vi "Get Dependencies.vi"(8 "error in":errorcluster, 9 "Entire Hierarchy":bool, 10 "File Path":path, 11 "LV File Creator in":refnum<class "LV File Creator.lvclass">) -> (0 "error out":errorcluster, 2 "Dependencies":path[](array[path]), 3 "LV File Creator out":refnum<class "LV File Creator.lvclass">)   [LabVIEW 2026, in "LV File Creator.lvclass"]
doc: "This VI determines dependencies of a LabVIEW file."
uses:
  LV File Creator.lvclass
  LV File Creator.lvclass/LV File Creator.ctl
  Interfaces/ILogger/ILogger Messages/Log Msg/Log Msg.lvclass
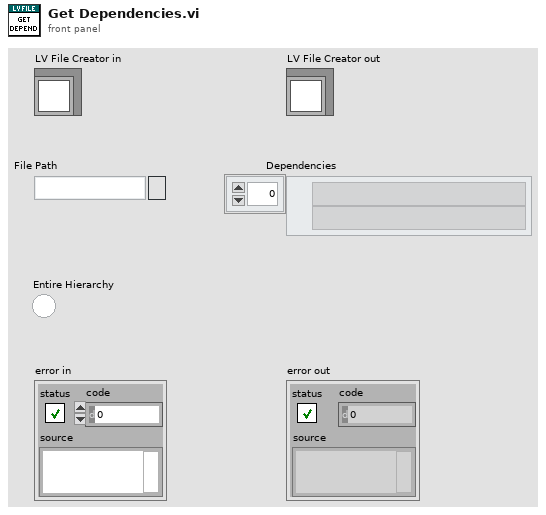
[diagram p1: front panel]
types:
  T1 = enum8{"Only include commented out diagrams if diagram already loaded", "Never include commented out diagrams", "Always include commented out diagrams"}
  T2 = typedef "Log Entry--cluster.ctl" = cluster{"Time":timestamp, "Message":string}
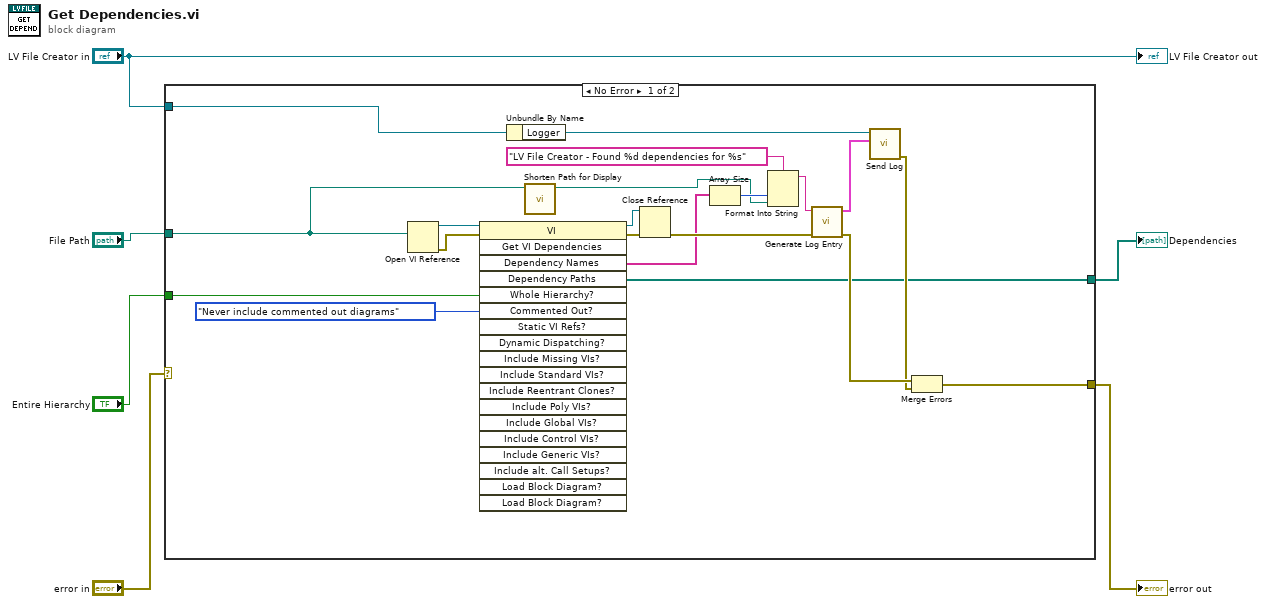
[diagram p0: block diagram]
diagram:
  n1 = case shown="No Error" "error in" {
    selector: "error in" -> [_ w27]
    tunnel: "LV File Creator in" -> [w20 _]
    tunnel: "File Path" -> [w14 _]
    tunnel: [w22 w27] -> w5
    tunnel: [w9 _] -> w2
    tunnel: "Entire Hierarchy" -> [w7 _]
    frame No Error {
      n2 = Open VI Reference(vi path=w14) -> (vi reference=w19:refnum<vi>, error out=w26:errorcluster)  [unwired: 5 in]
      n3 = invoke class="VI" method="Get VI Dependencies"(reference=w19, error in=w26, "Whole Hierarchy?"=w7, "Commented Out?"=T1."Never include commented out diagrams" ("Commented Out Diagrams?")) -> (reference out=w18:refnum<vi>, error out=w25:errorcluster, "Dependency Names"=w12:string[], "Dependency Paths"=w9:path[])  [unwired: 15 in, 15 out]
      n4 = Unbundle By Name(w20) -> ("Logger"=w17:refnum<class "Message Enqueuer.lvclass">)
      n5 = call "Shorten Path for Display.vi"("Path"=w14) -> ("Shortened Path"=w10:path)  [unwired: 10 in]
      n6 = Close Reference(reference=w18, error in (no error)=w25) -> (error out=w24:errorcluster)
      n7 = Array Size(array=w12) -> (size(s)=w11:i32)
      n8 = Format Into String(format string="LV File Creator - Found %d dependencies for %s", w11, w10) -> (resulting string=w13:string)  [unwired: 2 in, 1 out]
      n9 = call "Generate Log Entry.vi"("error in"=w24, "Message"=w13) -> ("error out"=w23:errorcluster, "Log Entry"=w16:T2)  [unwired: 8 in]
      n10 = call "Send Log.vi"("Log Entry"=w16, "Message Enqueuer"=w17) -> ("error out"=w21:errorcluster)  [unwired: 8 in, 1 out]
      n11 = Merge Errors(w23, w21) -> (w22:errorcluster)
    }
    frame Error {
      # "Pass error without further action."
    }
  }
  "error out" <- w5
  "Dependencies" <- w2
  "LV File Creator out" <- "LV File Creator in"
